vi "子VI-WriteSimple.vi"(2 "指令":string, 3 "超时":u32, 4 "会话":u32) -> (0 "描述":string, 1 "返回值":i32)   [LabVIEW 2011]
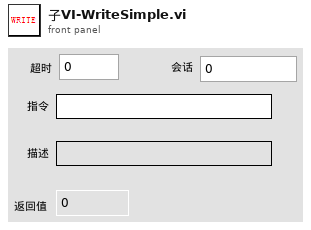
[diagram p1: front panel]
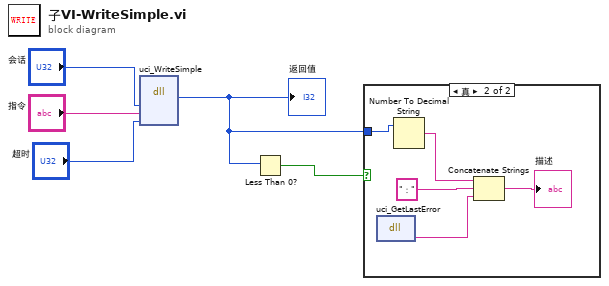
[diagram p0: block diagram]
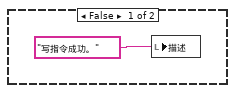
[diagram p2: hidden frame]
diagram:
  n1 = dll-call lib="PTH1Eabs E调试程序\nLabView程序UCI示例程序ASCIIuci.dll" fn="uci_WriteSimple"("session"="会话", "msg"="指令", "timeout"="超时") -> ("返回类型"=w1:i32)  [unwired: 6 in, 2 out]
  "返回值" <- w1
  n2 = Less Than 0?(x=w1) -> (x < 0?=w2:bool)
  n3 = case shown="真" w2 {
    tunnel: w1 -> [_ w8]
    frame False {
      n4 = local write "描述"("写指令成功。") -> ()
    }
    frame True {
      n5 = dll-call lib="PTH1Eabs E调试程序\nLabView程序UCI示例程序ASCIIuci.dll" fn="uci_GetLastError"() -> ("返回类型"=w9:string)  [unwired: 3 in, 2 out]
      n6 = Number To Decimal String(number=w8) -> (decimal integer string=w11:string)  [unwired: 1 in]
      n7 = Concatenate Strings(w11, "：", w9) -> (→"描述":string)
    }
  }
